vi "Emergancy Switch .vi"(8 "error in":errorcluster) -> (0 "error out":errorcluster, 1 "Command Response 2":string, 2 "Result":string, 3 "Pressed":bool)   [LabVIEW 2021]
uses:
  DUT/DUT_Cmd.ctl
panel:
  out "Result":bool
  out "number 2":dbl
  out "Pressed 2":bool
  out "number":dbl
  out "Command Response":string
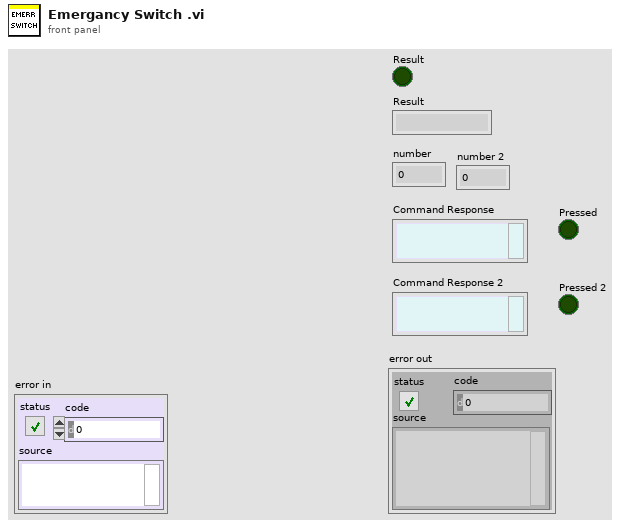
[diagram p1: front panel]
types:
  T1 = typedef "DUT_Cmd.ctl" = enum16{"Unlock serial", "Stop console logs", "Release emergency at start", "Read firmware", "WiFi credentials", "WiFi connected", "WiFi SSID", "Board revision", "ADC_NTC_TEMP", "ADC_TYPE2_RCD_CURRENT", "PCBA serial write", "PCBA serial readback", "Start energy meter", "Energy meter Vac", "Energy meter Iac", "Energy meter PF", "Energy meter energy", "Provision", "Set gateway identity", "CP checklist", "Earth detect", "D+M sense unplugged", "D+M sense plugged", "Output relay weld", "Start diagnostics", "Relay 1 on", "Relay 2 on", "Emergency pressed", "Release emergency", "Emergency released", "Unlock serial for 5 A", "Board current (5 A)", "Unlock serial for 15 A", "Board current (15 A)", "Unlock serial for 0 A", "NFC tag", "Start diagnostics again", "Relay 2 off", "Relay 1 off", "End diagnostics", "Load current (5 A) [No USB station]", "Load current (15 A) [No USB station]", "Load current (0 A) [No USB station]", "NFC tag [No USB station]", "Battery Voltage", "FW Power reset", "Notification LED", "O/P Relay weld Detection", "Earth Detection", "12V ", "5V", "3.3V", "Reboot"}
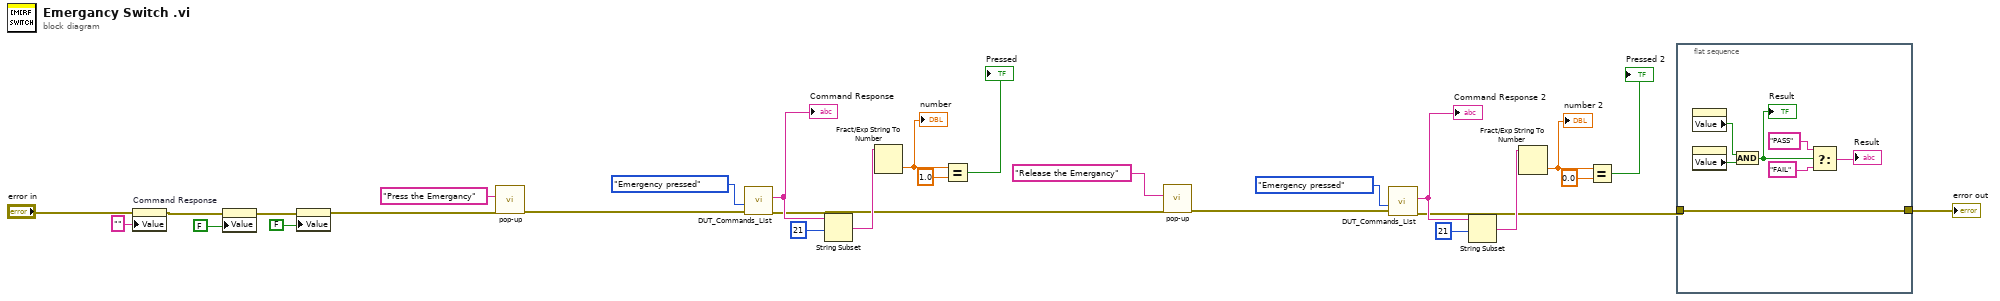
[diagram p0: block diagram]
diagram:
  n1 = property on="Command Response" class="Str"(error in="error in", "Value"="" ("Command Response")) -> (error out=w9:errorcluster)  [unwired: 1 in, 1 out]
  n2 = property on="Pressed" class="Bool (strict)"(error in=w9, "Value"=FALSE ("Pressed")) -> (error out=w10:errorcluster)  [unwired: 1 in, 1 out]
  n3 = property on="Pressed 2" class="Bool (strict)"(error in=w10, "Value"=FALSE ("Pressed 2")) -> (error out=w6:errorcluster)  [unwired: 1 in, 1 out]
  n4 = call "pop-up.vi"("error in"=w6, "input string"="Press the Emergancy") -> ("error out"=w5:errorcluster)  [unwired: 7 in, 2 out]
  n5 = call "DUT_Commands_List.vi"("error in"=w5, "DUT Cmd"=DUT_Cmd."Emergency pressed") -> ("error out"=w2:errorcluster, "Command Response"=w25:string)  [unwired: 7 in, 1 out]
  "Command Response" <- w25
  n6 = String Subset(string=w25, offset (0)=21) -> (substring=w23:string)  [unwired: 1 in]
  n7 = Fract/Exp String To Number(string=w23) -> (number=w22:dbl)  [unwired: 3 in, 1 out]
  "number" <- w22
  n8 = Equal?(x=w22, y=1.0) -> (x = y?=→"Pressed":bool)
  n9 = call "pop-up.vi"("error in"=w2, "input string"="Release the Emergancy") -> ("error out"=w1:errorcluster)  [unwired: 7 in, 2 out]
  n10 = call "DUT_Commands_List.vi"("error in"=w1, "DUT Cmd"=DUT_Cmd."Emergency pressed") -> ("error out"=w12:errorcluster, "Command Response"=w18:string)  [unwired: 7 in, 1 out]
  "Command Response 2" <- w18
  n11 = String Subset(string=w18, offset (0)=21) -> (substring=w16:string)  [unwired: 1 in]
  n12 = Fract/Exp String To Number(string=w16) -> (number=w15:dbl)  [unwired: 3 in, 1 out]
  "number 2" <- w15
  n13 = Equal?(x=w15, y=0.0) -> (x = y?=→"Pressed 2":bool)
  n14 = flat-sequence {
    tunnel: w12 -> [w29]
    tunnel: [w29] -> w11
    frame #0 {
      n15 = property on="Pressed" class="Bool (strict)"() -> ("Value"=w33:bool)  [unwired: 2 in, 2 out]
      n16 = property on="Pressed 2" class="Bool (strict)"() -> ("Value"=w34:bool)  [unwired: 2 in, 2 out]
      n17 = And(x=w33, y=w34) -> (x .and. y?=w35:bool)
      "Result" <- w35
      n18 = Select(t="PASS", s=w35, f="FAIL") -> (s? t:f=→"Result":string)
    }
  }
  "error out" <- w11
